vi "RemoteVI Check Window Rows.vi"() -> (4 "labels":string[](array[string]), 6 "expected":string[](array[string]), 8 "actual":string[](array[string]), 10 "failures":i32)   [LabVIEW 2020]
doc: "Test support, generated by tests/caraya/build.py from tests/vectors/server-app.json (windowRows) - do not edit. Calls RemoteVI Window Rows.vi once per vector: raw, labview only? and skip as in the vector; each row is rendered group|program|title|pid|hWnd with a line feed after it. Outputs, one element per vector: labels (the vector's name), expected (rendered from the vector), actual (the VI's result rendered the same way), and failures, the number of vectors whose expected and actual differ."
uses:
  source/RemoteVI.lvlib
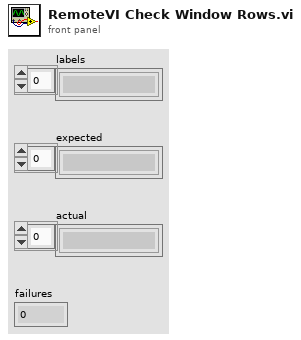
[diagram p1: front panel]
types:
  T1 = cluster{"name":string, "raw":cluster{"hWnd":u64, "pid":u32, "path":string, "class":string, "title":string, "visible":bool, "owned":bool, "ex style":u32, "w":i32, "h":i32}[], "lvo":bool, "skip":u64, "expect":string}[]
  T2 = cluster{"hWnd":u64, "pid":u32, "path":string, "class":string, "title":string, "visible":bool, "owned":bool, "ex style":u32, "w":i32, "h":i32}[]
  T3 = cluster{"group":i32, "program":string, "title":string, "pid":u32, "hWnd":u64}[]
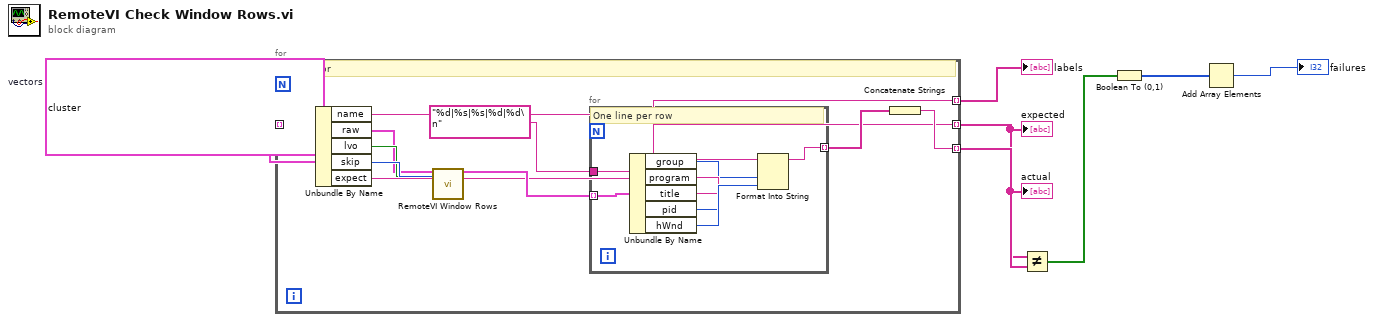
[diagram p0: block diagram]
diagram:
  w1 = T1 [{"name"="all programs", "raw"=[{"hWnd"=1001, "pid"=4000, "path"="C:\\Windows\\notepad.exe", "class"="Notepad", "title"="notes.txt - Notepad", "visible"=TRUE, "owned"=FALSE, "ex style"=0, "w"=400, "h"=300}, {"hWnd"=1002, "pid"=5000, "path"="C:\\Program Files\\National Instruments\\LabVIEW 2025\\LabVIEW.exe", "class"="LVDChild", "title"="RemoteVI Demo.vi", "visible"=TRUE, "owned"=TRUE, "ex style"=0, "w"=400, "h"=300}, {"hWnd"=1003, "pid"=5000, "path"="C:\\Program Files\\National Instruments\\LabVIEW 2025\\LabVIEW.exe", "class"="LVDChild", "title"="RemoteVI Demo.vi Block Diagram", "visible"=TRUE, "owned"=TRUE, "ex style"=0, "w"=400, "h"=300}, {"hWnd"=1004, "pid"=5000, "path"="C:\\Program Files\\National Instruments\\LabVIEW 2025\\LabVIEW.exe", "class"="LVDChild", "title"="RemoteVI.lvproj - Project Explorer", "visible"=TRUE, "owned"=TRUE, "ex style"=0, "w"=400, "h"=300}, {"hWnd"=1005, "pid"=6000, "path"="D:\\apps\\Test Stand.exe", "class"="LVDChild", "title"="Main.vi", "visible"=TRUE, "owned"=TRUE, "ex style"=0, "w"=400, "h"=300}, {"hWnd"=1006, "pid"=4000, "path"="C:\\Windows\\notepad.exe", "class"="#32770", "title"="Save As", "visible"=TRUE, "owned"=TRUE, "ex style"=0, "w"=400, "h"=300}, {"hWnd"=1007, "pid"=7000, "path"="C:\\Windows\\explorer.exe", "class"="Shell_TrayWnd", "title"="", "visible"=TRUE, "owned"=FALSE, "ex style"=0, "w"=400, "h"=300}, {"hWnd"=1008, "pid"=7000, "path"="C:\\Windows\\explorer.exe", "class"="CabinetWClass", "title"="Documents", "visible"=FALSE, "owned"=FALSE, "ex style"=0, "w"=400, "h"=300}, {"hWnd"=1009, "pid"=8000, "path"="C:\\tools\\Calc.exe", "class"="ApplicationFrameWindow", "title"="Calculator", "visible"=TRUE, "owned"=FALSE, "ex style"=0, "w"=400, "h"=300}, {"hWnd"=1010, "pid"=8000, "path"="C:\\tools\\Calc.exe", "class"="Tip", "title"="tool tip", "visible"=TRUE, "owned"=FALSE, "ex style"=128, "w"=400, "h"=300}, {"hWnd"=1011, "pid"=5000, "path"="C:\\Program Files\\National Instruments\\LabVIEW 2025\\LabVIEW.exe", "class"="LVDChild", "title"="A first.vi", "visible"=TRUE, "owned"=TRUE, "ex style"=0, "w"=400, "h"=300}, {"hWnd"=1012, "pid"=5000, "path"="C:\\Program Files\\National Instruments\\LabVIEW 2025\\LabVIEW.exe", "class"="LVDChild", "title"="RemoteVI Server", "visible"=TRUE, "owned"=TRUE, "ex style"=0, "w"=400, "h"=300}, {"hWnd"=1013, "pid"=9000, "path"="C:\\x\\zero.exe", "class"="Zero", "title"="zero size", "visible"=TRUE, "owned"=FALSE, "ex style"=0, "w"=0, "h"=300}, {"hWnd"=1014, "pid"=9100, "path"="C:\\Windows\\TextInputHost.exe", "class"="Windows.UI.Core.CoreWindow", "title"="Input experience", "visible"=TRUE, "owned"=FALSE, "ex style"=0, "w"=400, "h"=300}, {"hWnd"=1015, "pid"=9200, "path"="C:\\x\\small.exe", "class"="Small", "title"="tiny window", "visible"=TRUE, "owned"=FALSE, "ex style"=0, "w"=99, "h"=300}, {"hWnd"=1016, "pid"=9300, "path"="C:\\x\\overlay.exe", "class"="Ovl", "title"="no activate", "visible"=TRUE, "owned"=FALSE, "ex style"=134217728, "w"=400, "h"=300}], "lvo"=FALSE, "skip"=1012, "expect"="0|LabVIEW.exe|A first.vi|5000|1011\n0|LabVIEW.exe|RemoteVI Demo.vi|5000|1002\n1|Test Stand.exe|Main.vi|6000|1005\n2|Calc.exe|Calculator|8000|1009\n2|notepad.exe|notes.txt - Notepad|4000|1001\n"}, {"name"="LabVIEW only", "raw"=[{"hWnd"=1001, "pid"=4000, "path"="C:\\Windows\\notepad.exe", "class"="Notepad", "title"="notes.txt - Notepad", "visible"=TRUE, "owned"=FALSE, "ex style"=0, "w"=400, "h"=300}, {"hWnd"=1002, "pid"=5000, "path"="C:\\Program Files\\National Instruments\\LabVIEW 2025\\LabVIEW.exe", "class"="LVDChild", "title"="RemoteVI Demo.vi", "visible"=TRUE, "owned"=TRUE, "ex style"=0, "w"=400, "h"=300}, {"hWnd"=1003, "pid"=5000, "path"="C:\\Program Files\\National Instruments\\LabVIEW 2025\\LabVIEW.exe", "class"="LVDChild", "title"="RemoteVI Demo.vi Block Diagram", "visible"=TRUE, "owned"=TRUE, "ex style"=0, "w"=400, "h"=300}, {"hWnd"=1004, "pid"=5000, "path"="C:\\Program Files\\National Instruments\\LabVIEW 2025\\LabVIEW.exe", "class"="LVDChild", "title"="RemoteVI.lvproj - Project Explorer", "visible"=TRUE, "owned"=TRUE, "ex style"=0, "w"=400, "h"=300}, {"hWnd"=1005, "pid"=6000, "path"="D:\\apps\\Test Stand.exe", "class"="LVDChild", "title"="Main.vi", "visible"=TRUE, "owned"=TRUE, "ex style"=0, "w"=400, "h"=300}, {"hWnd"=1006, "pid"=4000, "path"="C:\\Windows\\notepad.exe", "class"="#32770", "title"="Save As", "visible"=TRUE, "owned"=TRUE, "ex style"=0, "w"=400, "h"=300}, {"hWnd"=1007, "pid"=7000, "path"="C:\\Windows\\explorer.exe", "class"="Shell_TrayWnd", "title"="", "visible"=TRUE, "owned"=FALSE, "ex style"=0, "w"=400, "h"=300}, {"hWnd"=1008, "pid"=7000, "path"="C:\\Windows\\explorer.exe", "class"="CabinetWClass", "title"="Documents", "visible"=FALSE, "owned"=FALSE, "ex style"=0, "w"=400, "h"=300}, {"hWnd"=1009, "pid"=8000, "path"="C:\\tools\\Calc.exe", "class"="ApplicationFrameWindow", "title"="Calculator", "visible"=TRUE, "owned"=FALSE, "ex style"=0, "w"=400, "h"=300}, {"hWnd"=1010, "pid"=8000, "path"="C:\\tools\\Calc.exe", "class"="Tip", "title"="tool tip", "visible"=TRUE, "owned"=FALSE, "ex style"=128, "w"=400, "h"=300}, {"hWnd"=1011, "pid"=5000, "path"="C:\\Program Files\\National Instruments\\LabVIEW 2025\\LabVIEW.exe", "class"="LVDChild", "title"="A first.vi", "visible"=TRUE, "owned"=TRUE, "ex style"=0, "w"=400, "h"=300}, {"hWnd"=1012, "pid"=5000, "path"="C:\\Program Files\\National Instruments\\LabVIEW 2025\\LabVIEW.exe", "class"="LVDChild", "title"="RemoteVI Server", "visible"=TRUE, "owned"=TRUE, "ex style"=0, "w"=400, "h"=300}, {"hWnd"=1013, "pid"=9000, "path"="C:\\x\\zero.exe", "class"="Zero", "title"="zero size", "visible"=TRUE, "owned"=FALSE, "ex style"=0, "w"=0, "h"=300}, {"hWnd"=1014, "pid"=9100, "path"="C:\\Windows\\TextInputHost.exe", "class"="Windows.UI.Core.CoreWindow", "title"="Input experience", "visible"=TRUE, "owned"=FALSE, "ex style"=0, "w"=400, "h"=300}, {"hWnd"=1015, "pid"=9200, "path"="C:\\x\\small.exe", "class"="Small", "title"="tiny window", "visible"=TRUE, "owned"=FALSE, "ex style"=0, "w"=99, "h"=300}, {"hWnd"=1016, "pid"=9300, "path"="C:\\x\\overlay.exe", "class"="Ovl", "title"="no activate", "visible"=TRUE, "owned"=FALSE, "ex style"=134217728, "w"=400, "h"=300}], "lvo"=TRUE, "skip"=1012, "expect"="0|LabVIEW.exe|A first.vi|5000|1011\n0|LabVIEW.exe|RemoteVI Demo.vi|5000|1002\n1|Test Stand.exe|Main.vi|6000|1005\n"}, {"name"="nothing skipped", "raw"=[{"hWnd"=1001, "pid"=4000, "path"="C:\\Windows\\notepad.exe", "class"="Notepad", "title"="notes.txt - Notepad", "visible"=TRUE, "owned"=FALSE, "ex style"=0, "w"=400, "h"=300}, {"hWnd"=1002, "pid"=5000, "path"="C:\\Program Files\\National Instruments\\LabVIEW 2025\\LabVIEW.exe", "class"="LVDChild", "title"="RemoteVI Demo.vi", "visible"=TRUE, "owned"=TRUE, "ex style"=0, "w"=400, "h"=300}, {"hWnd"=1003, "pid"=5000, "path"="C:\\Program Files\\National Instruments\\LabVIEW 2025\\LabVIEW.exe", "class"="LVDChild", "title"="RemoteVI Demo.vi Block Diagram", "visible"=TRUE, "owned"=TRUE, "ex style"=0, "w"=400, "h"=300}, {"hWnd"=1004, "pid"=5000, "path"="C:\\Program Files\\National Instruments\\LabVIEW 2025\\LabVIEW.exe", "class"="LVDChild", "title"="RemoteVI.lvproj - Project Explorer", "visible"=TRUE, "owned"=TRUE, "ex style"=0, "w"=400, "h"=300}, {"hWnd"=1005, "pid"=6000, "path"="D:\\apps\\Test Stand.exe", "class"="LVDChild", "title"="Main.vi", "visible"=TRUE, "owned"=TRUE, "ex style"=0, "w"=400, "h"=300}, {"hWnd"=1006, "pid"=4000, "path"="C:\\Windows\\notepad.exe", "class"="#32770", "title"="Save As", "visible"=TRUE, "owned"=TRUE, "ex style"=0, "w"=400, "h"=300}, {"hWnd"=1007, "pid"=7000, "path"="C:\\Windows\\explorer.exe", "class"="Shell_TrayWnd", "title"="", "visible"=TRUE, "owned"=FALSE, "ex style"=0, "w"=400, "h"=300}, {"hWnd"=1008, "pid"=7000, "path"="C:\\Windows\\explorer.exe", "class"="CabinetWClass", "title"="Documents", "visible"=FALSE, "owned"=FALSE, "ex style"=0, "w"=400, "h"=300}, {"hWnd"=1009, "pid"=8000, "path"="C:\\tools\\Calc.exe", "class"="ApplicationFrameWindow", "title"="Calculator", "visible"=TRUE, "owned"=FALSE, "ex style"=0, "w"=400, "h"=300}, {"hWnd"=1010, "pid"=8000, "path"="C:\\tools\\Calc.exe", "class"="Tip", "title"="tool tip", "visible"=TRUE, "owned"=FALSE, "ex style"=128, "w"=400, "h"=300}, {"hWnd"=1011, "pid"=5000, "path"="C:\\Program Files\\National Instruments\\LabVIEW 2025\\LabVIEW.exe", "class"="LVDChild", "title"="A first.vi", "visible"=TRUE, "owned"=TRUE, "ex style"=0, "w"=400, "h"=300}, {"hWnd"=1012, "pid"=5000, "path"="C:\\Program Files\\National Instruments\\LabVIEW 2025\\LabVIEW.exe", "class"="LVDChild", "title"="RemoteVI Server", "visible"=TRUE, "owned"=TRUE, "ex style"=0, "w"=400, "h"=300}, {"hWnd"=1013, "pid"=9000, "path"="C:\\x\\zero.exe", "class"="Zero", "title"="zero size", "visible"=TRUE, "owned"=FALSE, "ex style"=0, "w"=0, "h"=300}, {"hWnd"=1014, "pid"=9100, "path"="C:\\Windows\\TextInputHost.exe", "class"="Windows.UI.Core.CoreWindow", "title"="Input experience", "visible"=TRUE, "owned"=FALSE, "ex style"=0, "w"=400, "h"=300}, {"hWnd"=1015, "pid"=9200, "path"="C:\\x\\small.exe", "class"="Small", "title"="tiny window", "visible"=TRUE, "owned"=FALSE, "ex style"=0, "w"=99, "h"=300}, {"hWnd"=1016, "pid"=9300, "path"="C:\\x\\overlay.exe", "class"="Ovl", "title"="no activate", "visible"=TRUE, "owned"=FALSE, "ex style"=134217728, "w"=400, "h"=300}], "lvo"=TRUE, "skip"=0, "expect"="0|LabVIEW.exe|A first.vi|5000|1011\n0|LabVIEW.exe|RemoteVI Demo.vi|5000|1002\n0|LabVIEW.exe|RemoteVI Server|5000|1012\n1|Test Stand.exe|Main.vi|6000|1005\n"}]  # vectors
  n1 = for {
    tunnel: w1 -> [w8] mode=indexing
    tunnel: [w9] -> w2 mode=indexing
    tunnel: [w13] -> w3 mode=indexing
    tunnel: [w17] -> w4 mode=indexing
    # "One vector"
    n2 = Unbundle By Name(w8) -> ("name"=w9:string, "raw"=w10:T2, "lvo"=w11:bool, "skip"=w12:u64, "expect"=w13:string)
    n3 = call "RemoteVI Window Rows.vi"("raw"=w10, "labview only?"=w11, "skip"=w12) -> ("rows"=w14:T3)  [unwired: 12 in]
    n4 = for {
      tunnel: "%d|%s|%s|%d|%d\n" -> [w19]
      tunnel: w14 -> [w18] mode=indexing
      tunnel: [w25] -> w16 mode=indexing
      # "One line per row"
      n5 = Unbundle By Name(w18) -> ("group"=w20:i32, "program"=w21:string, "title"=w22:string, "pid"=w23:u32, "hWnd"=w24:u64)
      n6 = Format Into String(format string=w19, w20, w21, w22, w23, w24) -> (resulting string=w25:string)  [unwired: 2 in, 1 out]
    }
    n7 = Concatenate Strings(w16) -> (w17:string)
  }
  "labels" <- w2
  "expected" <- w3
  "actual" <- w4
  n8 = Not Equal?(x=w3, y=w4) -> (x != y?=w5:bool[])
  n9 = Boolean To (0,1)(Boolean=w5) -> (0, 1=w6:i16[])
  n10 = Add Array Elements(numeric array=w6) -> (sum=→"failures":i16)
